vi "Update Message Setter.vi"(7 "rpc message name":string, 8 "error in (no error)":errorcluster, 10 "message setter in":refnum<vi>, 11 "rpc messages folder in":refnum<vi>) -> (0 "error out":errorcluster, 2 "message setter out":refnum<vi>, 3 "rpc messages folder out":refnum<vi>)   [LabVIEW 2019, in "gRPC Template Creation Utility.lvlib"]
uses:
  gRPC Template Creation Utility.lvlib
  Oneof API/OneOf Constants/OneOfConstantsEnum.ctl
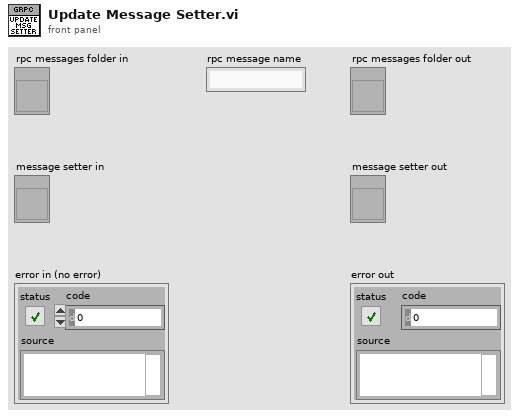
[diagram p1: front panel]
types:
  T1 = typedef "gRPC Template Creation Utility.lvlib/OneOfConstantsEnum.ctl" = enum16{"FlatToRichVIPrefix", "RichToFlatVIPrefix", "FlatTypeDefSuffix"}
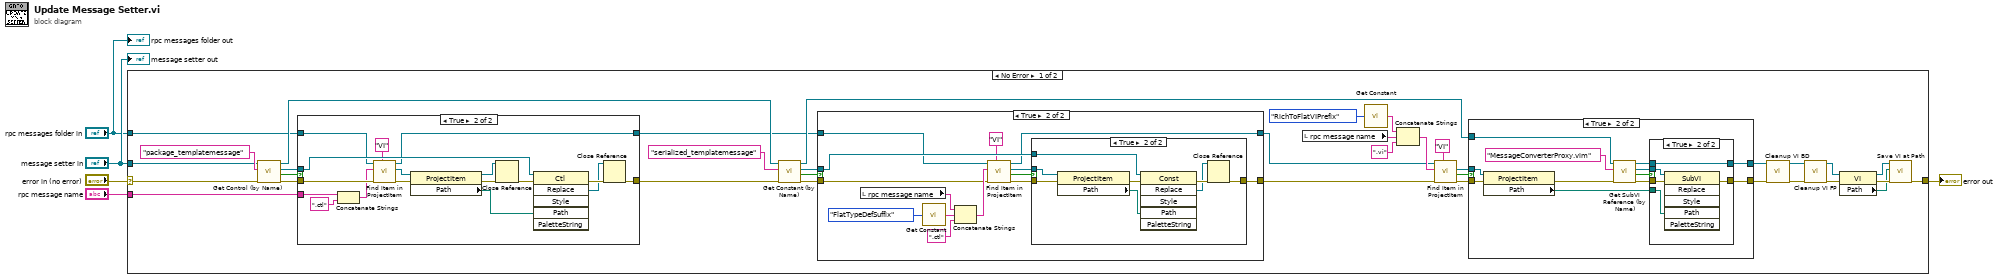
[diagram p0: block diagram]
diagram:
  n1 = case shown="No Error" "error in (no error)" {
    selector: "error in (no error)" -> [w16 w108]
    tunnel: "message setter in" -> [w17 _]
    tunnel: [w13 w108] -> w4
    tunnel: "rpc message name" -> [w12 _]
    tunnel: "rpc messages folder in" -> [w15 _]
    frame No Error {
      n2 = call "Get Control (by Name).vi"("error in (no error)"=w16, "Control Label"="package_templatemessage" ("name/order"), "Owner VI in"=w17) -> ("error out"=w41:errorcluster, "Found ?"=w42:bool, "Control Refnum"=w40:refnum<vi>, "Owner VI out"=w39:refnum<vi>)  [unwired: 5 in]
      n3 = case shown="True" w42 {
        tunnel: [w90 w107] -> w26
        tunnel: w40 -> [_ w104]
        tunnel: w41 -> [w90 w95]
        tunnel: w15 -> [w89 w98]
        tunnel: [w89 w97] -> w14
        tunnel: w12 -> [_ w93]
        frame False {
        }
        frame True {
          n4 = Concatenate Strings(w93, ".ctl" ("string")) -> (w91:string)
          n5 = call "Find Item in ProjectItem.vi"("Item Type"="VI", "error in (no error)"=w95, "Name"=w91, "ProjectItem in"=w98) -> ("error out"=w102:errorcluster, "Item Refnum out"=w103:refnum<vi>, "ProjectItem out"=w97:refnum<vi>)  [unwired: 4 in, 1 out]
          n6 = property class="ProjectItem"(reference=w103, error in=w102) -> (reference out=w101:refnum<vi>, error out=w100:errorcluster, "Path"=w96:path)
          n7 = Close Reference(reference=w101, error in (no error)=w100) -> (error out=w94:errorcluster)
          n8 = invoke class="Ctl" method="Replace"(reference=w104, error in=w94, "Path"=w96) -> (error out=w106:errorcluster, "Replace"=w105:refnum<vi>)  [unwired: 3 in, 4 out]
          n9 = Close Reference(reference=w105, error in (no error)=w106) -> (error out=w107:errorcluster)
        }
      }
      n10 = call "Get Constant (by Name).vi"("error in (no error)"=w26, "Constant Label"="serialized_templatemessage", "Owner VI in"=w39) -> ("error out"=w35:errorcluster, "Found ?"=w36:bool, "Const ref out"=w37:refnum<vi>, "Owner VI out"=w33:refnum<vi>)  [unwired: 5 in]
      n11 = case shown="True" w36 {
        tunnel: [w65 w79] -> w25
        tunnel: w37 -> [_ w78]
        tunnel: w35 -> [w65 w68]
        tunnel: w14 -> [w64 w75]
        tunnel: [w64 w72] -> w24
        frame False {
        }
        frame True {
          n12 = local read "rpc message name"() -> (w77:string)
          n13 = call "Get Constant.vi"("Selection"=OneOfConstantsEnum."FlatTypeDefSuffix") -> ("String"=w66:string)
          n14 = Concatenate Strings(w77, w66, ".ctl" ("string")) -> (w74:string)
          n15 = call "Find Item in ProjectItem.vi"("Item Type"="VI", "error in (no error)"=w68, "Name"=w74, "ProjectItem in"=w75) -> ("error out"=w69:errorcluster, "Found ?"=w70:bool, "Item Refnum out"=w71:refnum<vi>, "ProjectItem out"=w72:refnum<vi>)  [unwired: 4 in]
          n16 = case shown="True" w70 {
            tunnel: [w80 w88] -> w79
            tunnel: w78 -> [_ w85]
            tunnel: w71 -> [_ w84]
            tunnel: w69 -> [w80 w82]
            frame False {
            }
            frame True {
              n17 = property class="ProjectItem"(reference=w84, error in=w82) -> (error out=w81:errorcluster, "Path"=w83:path)  [unwired: 1 out]
              n18 = invoke class="Const" method="Replace"(reference=w85, error in=w81, "Path"=w83) -> (error out=w87:errorcluster, "Replace"=w86:refnum<vi>)  [unwired: 3 in, 4 out]
              n19 = Close Reference(reference=w86, error in (no error)=w87) -> (error out=w88:errorcluster)
            }
          }
        }
      }
      n20 = local read "rpc message name"() -> (w32:string)
      n21 = call "Get Constant.vi"("Selection"=OneOfConstantsEnum."RichToFlatVIPrefix") -> ("String"=w21:string)
      n22 = Concatenate Strings(w21, w32, ".vi" ("string")) -> (w30:string)
      n23 = call "Find Item in ProjectItem.vi"("Item Type"="VI", "error in (no error)"=w25, "Name"=w30, "ProjectItem in"=w24) -> ("error out"=w27:errorcluster, "Found ?"=w28:bool, "Item Refnum out"=w23:refnum<vi>)  [unwired: 4 in, 1 out]
      n24 = case shown="True" w28 {
        tunnel: w33 -> [w44 w56]
        tunnel: w27 -> [w43 w49]
        tunnel: [w43 w51] -> w9
        tunnel: [w44 w45] -> w7
        tunnel: w23 -> [_ w50]
        frame False {
        }
        frame True {
          n25 = property class="ProjectItem"(reference=w50, error in=w49) -> (error out=w48:errorcluster, "Path"=w47:path)  [unwired: 1 out]
          n26 = call "Get SubVI Reference (by Name).vi"("error in (no error)"=w48, "SubVI Name"="MessageConverterProxy.vim", "Owner VI in"=w56) -> ("error out"=w52:errorcluster, "Found ?"=w54:bool, "SubVI Refnum out"=w53:refnum<vi>, "Owner VI out"=w46:refnum<vi>)  [unwired: 5 in]
          n27 = case shown="True" w54 {
            tunnel: w53 -> [_ w63]
            tunnel: w52 -> [w58 w62]
            tunnel: [w58 w61] -> w51
            tunnel: w47 -> [_ w60]
            tunnel: w46 -> [w57 w59]
            tunnel: [w57 w59] -> w45
            frame False {
            }
            frame True {
              n28 = invoke class="SubVI" method="Replace"(reference=w63, error in=w62, "Path"=w60) -> (error out=w61:errorcluster)  [unwired: 3 in, 5 out]
            }
          }
        }
      }
      n29 = call "Cleanup VI BD.vi"("error in (no error)"=w9, "VI in"=w7) -> ("error out"=w11:errorcluster, "VI out"=w10:refnum<vi>)  [unwired: 8 in]
      n30 = call "Cleanup VI FP.vi"("error in"=w11, "vi in"=w10) -> ("error out"=w8:errorcluster, "vi out"=w6:refnum<vi>)  [unwired: 8 in]
      n31 = property class="VI"(reference=w6, error in=w8) -> (reference out=w20:refnum<vi>, error out=w19:errorcluster, "Path"=w18:path)
      n32 = call "Save VI at Path.vi"("error in (no error)"=w19, "Path"=w18, "VI in"=w20) -> ("error out"=w13:errorcluster)  [unwired: 6 in, 2 out]
    }
    frame Error {
    }
  }
  "error out" <- w4
  "rpc messages folder out" <- "rpc messages folder in"
  "message setter out" <- "message setter in"
